vi "Set AS7431.vi"(8 "error in (no error)":errorcluster, 11 "AS7431 Light Spectrum in":refnum<class "AS7431 11 Ch Light Spectrum Sensor.lvclass">) -> (0 "error out":errorcluster, 3 "AS7431 Light Spectrum out":refnum<class "AS7431 11 Ch Light Spectrum Sensor.lvclass">)   [LabVIEW 2020, in "CTI-Peripheral.lvlib" / "AS7431 11 Ch Light Spectrum Sensor.lvclass"]
uses:
  AS7431 11 Ch Light Spectrum Sensor.lvclass
  AS7431 11 Ch Light Spectrum Sensor.lvclass/AS7431 11 Ch Light Spectrum Sensor.ctl
  CTI/I2C Connection/I2C Connection.lvclass/I2C Connection.ctl
  CTI/Session/I2C Write Data.vi
  CTI/Session/I2C Read Data.vi
  CTI/I2C Connection/I2C Connection.lvclass
panel:
  out "Data":string
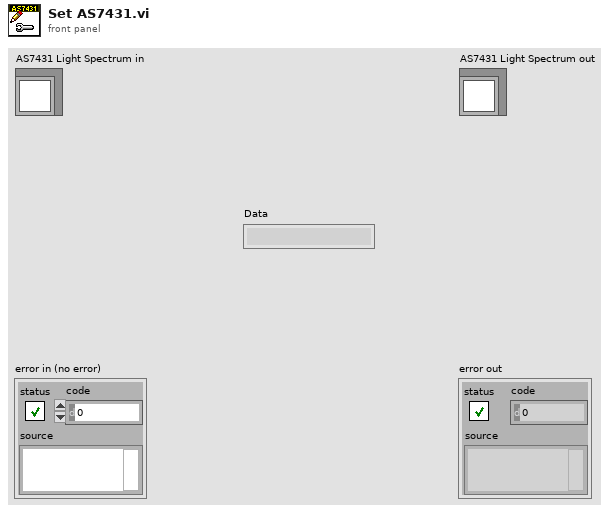
[diagram p1: front panel]
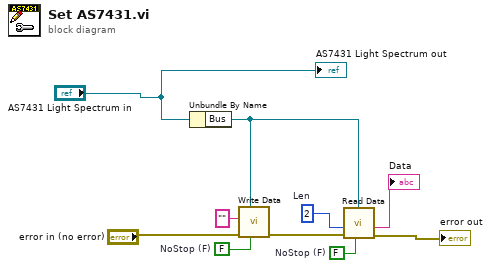
[diagram p0: block diagram]
diagram:
  w7 = FALSE  # NoStop (F)
  w8 = u8 2  # Len
  w9 = FALSE  # NoStop (F)
  n1 = Unbundle By Name("AS7431 Light Spectrum in") -> ("Bus"=w6:refnum<class "I2C Connection.lvclass">)
  n2 = call "Write Data.vi"("NoStop (F)"=w9, "I2C Connection"=w6, "error in (no error)"="error in (no error)", "Data"="") -> ("error out"=w5:errorcluster)  [unwired: 7 in]
  n3 = call "Read Data.vi"("NoStop (F)"=w7, "I2C Connection"=w6, "error in (no error)"=w5, "Len"=w8) -> ("error out"=→"error out":errorcluster, "Data"=→"Data":string)  [unwired: 6 in]
  "AS7431 Light Spectrum out" <- "AS7431 Light Spectrum in"
